vi "Measuring R with Agilent 34401A.vi"() -> ()   [LabVIEW 2018]
uses:
  <instrlib>/Agilent 34401/Public/Data/Read (Single Point).vi
  <instrlib>/Agilent 34401/Agilent 34401.lvlib
panel:
  in  "Function (0: DC Voltage)":u16(ring)=2 items=["DC Voltage", "AC Voltage", "2 - Wire Resistance", "4 - Wire Resistance", "DC Current", "AC Current", "Frequency", "Period", "Continuity", "Diode Checking", "VDC:VDC Ratio", "Temperature", "Capacitance"]
  in  "stop":bool
  out "Measurement":dbl format="%_6p"
  in  "VISA resource name":refnum<visa-resource-name>
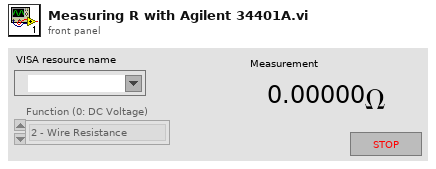
[diagram p1: front panel]
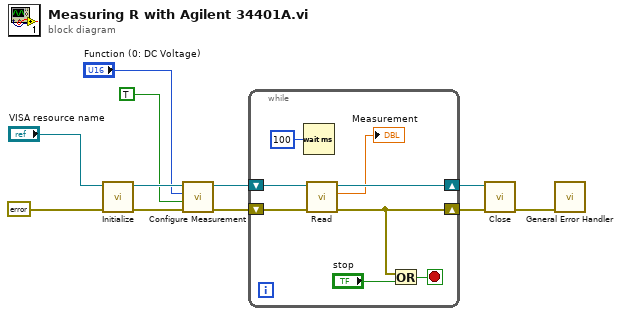
[diagram p0: block diagram]
diagram:
  n1 = call <instrlib>:"Initialize.vi"("error in (no error)"=errorcluster {"status"=FALSE, "code"=0, "source"=""}, "VISA resource name"="VISA resource name") -> ("error out"=w9:errorcluster, "VISA resource name out"=w8:refnum<visa-resource-name>)  [unwired: 8 in]
  n2 = call <instrlib>:"Configure Measurement.vi"("error in (no error)"=w9, "Enable Auto Range (T: Enable)"=TRUE, "Function (0: DC Voltage)"="Function (0: DC Voltage)", "VISA resource name"=w8) -> ("error out"=w2:errorcluster, "VISA resource name out"=w1:refnum<visa-resource-name>)  [unwired: 6 in]
  n3 = while {
    shift-right: [w12] -> w5
    shift-left: w2 -> [w19]
    shift-right: [w17] -> w6
    shift-left: w1 -> [w18]
    stop <- w13 stop-if-true
    n4 = Wait (ms)(milliseconds to wait=u32 100) -> ()  [unwired: 1 out]
    n5 = call-poly <instrlib>:"Read.vi"("error in (no error)"=w19, "VISA resource name"=w18) -> ("error out"=w12:errorcluster, "Measurement"=→"Measurement":dbl, "VISA resource name out"=w17:refnum<visa-resource-name>)  [unwired: 7 in]
    n6 = Or(x=w12, y="stop") -> (x .or. y?=w13:bool)
  }
  n7 = call <instrlib>:"Close.vi"("error in (no error)"=w5, "VISA resource name"=w6) -> ("error out"=w3:errorcluster)  [unwired: 9 in]
  n8 = call <vilib>:"General Error Handler.vi"("error in (no error)"=w3) -> ()  [unwired: 10 in, 5 out]
